vi "Open Modbus.vi"(8 "error in (no error)":errorcluster, 11 "Modbus_RTU in":refnum<class "Modbus_RTU.lvclass">) -> (0 "error out":errorcluster, 3 "Modbus_RTU out":refnum<class "Modbus_RTU.lvclass">)   [LabVIEW 2021, in "Modbus_RTU.lvclass"]
uses:
  Modbus_RTU.lvclass
  C:/Users/lincoln.lucio/Documents/Lincoln/Documentos Pessoais/meus docs/Projetos pessoais/Projeto Sciranda/projeto_versioned/sciranda/Modbus_Master/Modbus_Master.lvclass
  Modbus_Master/Modbus_Master.lvclass/Modbus_Master.ctl
  Modbus_RTU.lvclass/Modbus_RTU.ctl
  <vilib>/NI/Modbus Library/API/Modbus API.lvclass/Modbus API.ctl
  <vilib>/NI/Modbus Library/Transmission Data Unit/Transmission Data Unit.lvclass/Transmission Data Unit.ctl
  Modbus_Master/Accessor VIs/Read unit ID.vi
  Modbus_Master/Accessor VIs/Read Timeout(ms).vi
  <vilib>/NI/Modbus Library/API/Master/Set Write Timeout.vi
  Modbus_Master/Accessor VIs/Write master instance.vi
  <vilib>/NI/Modbus Library/API/Read Transmission Data Unit.vi
  <vilib>/NI/Modbus Library/API/Write Transmission Data Unit.vi
  <vilib>/NI/Modbus Library/Transmission Data Unit/Write write operation timeout.vi
  <vilib>/NI/Modbus Library/API/Master/Modbus Master.lvclass
  C:/Program Files/National Instruments/LabVIEW 2021/vi.lib/NI/Modbus Library/API/Modbus API.lvclass
  <vilib>/NI/Modbus Library/API/Wrapper/Create Serial Master.vi
  <vilib>/NI/Modbus Library/API/Wrapper/API Main.lvlib
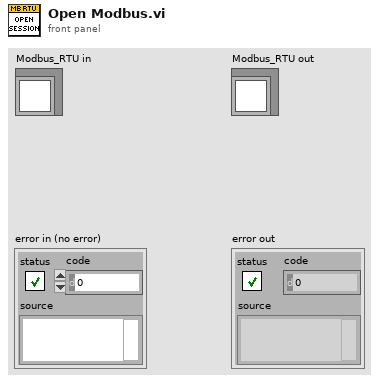
[diagram p1: front panel]
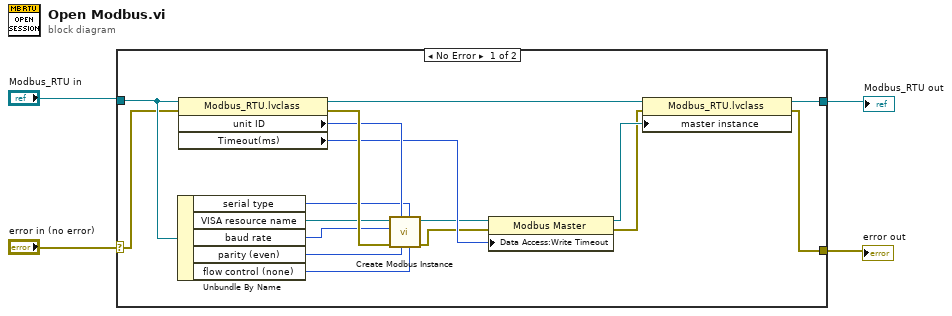
[diagram p0: block diagram]
diagram:
  n1 = case shown="No Error" "error in (no error)" {
    selector: "error in (no error)" -> [w16 w23]
    tunnel: [w21 w22] -> w3
    tunnel: "Modbus_RTU in" -> [w20 w22]
    tunnel: [w17 w23] -> w4
    frame No Error {
      n2 = Unbundle By Name(w20) -> ("serial type"=w12:enum16{"RTU", "ASCII"}, "VISA resource name"=w15:refnum<visa-resource-name>, "baud rate"=w13:u32, "parity (even)"=w11:u16, "flow control (none)"=w10:u16)
      n3 = property class="Modbus_RTU.lvclass"(reference=w20, error in=w16) -> (reference out=w19:refnum<class "Modbus_RTU.lvclass">, error out=w18:errorcluster, "unit ID"=w14:u8, "Timeout(ms)"=w9:i32)
      n4 = call-poly <vilib>:"Create Modbus Instance.vi"("flow control (none)"=w10, "serial type"=w12, "parity (even)"=w11, "unit ID"=w14, "error in"=w18, "baud rate"=w13, "VISA resource name"=w15) -> ("error out"=w7:errorcluster, "serial master instance"=w8:refnum<class "Modbus Master.lvclass">)  [unwired: 3 in]
      n5 = property class="Modbus Master"(reference=w8, error in=w7, "Data Access:Write Timeout"=w9) -> (reference out=w6:refnum<class "Modbus Master.lvclass">, error out=w5:errorcluster)
      n6 = property class="Modbus_RTU.lvclass"(reference=w19, error in=w5, "master instance"=w6) -> (reference out=w21:refnum<class "Modbus_RTU.lvclass">, error out=w17:errorcluster)
    }
    frame Error {
    }
  }
  "error out" <- w4
  "Modbus_RTU out" <- w3
